vi "ConvertErrorToPLCMBits.vi"(11 "Error message":string) -> (2 "PLC message":string, 3 "Send?":bool)   [LabVIEW 2025]
uses:
  <vilib>/Utility/error.llb/Trim Whitespace One-Sided.vi
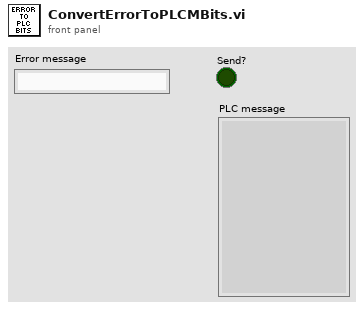
[diagram p1: front panel]
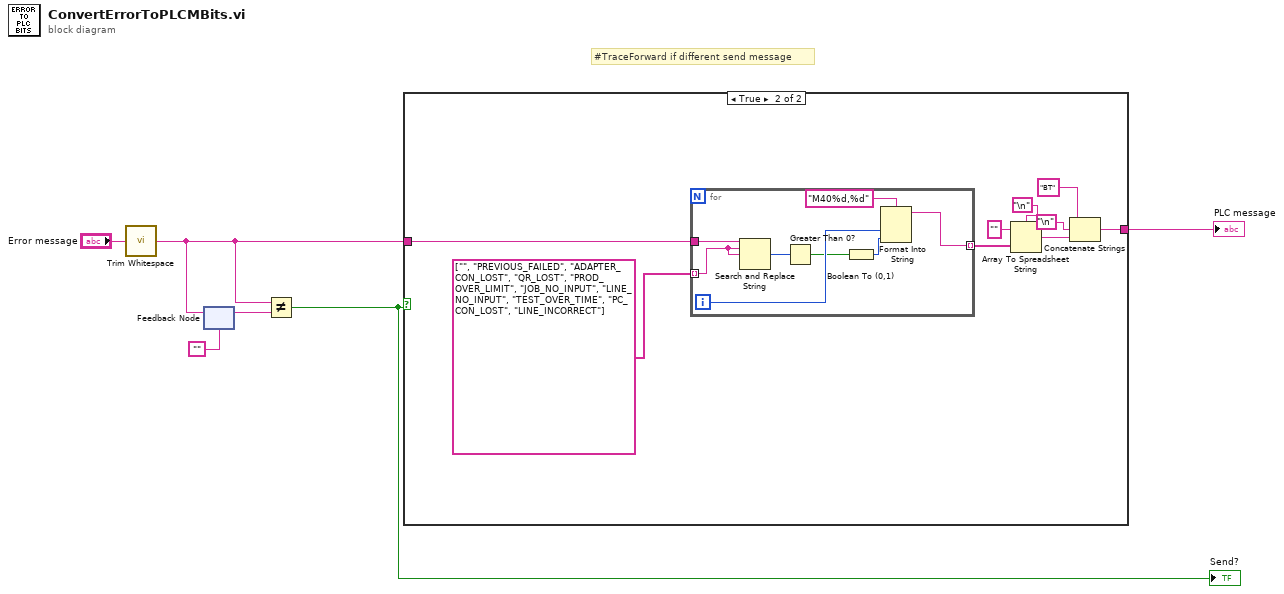
[diagram p0: block diagram]
diagram:
  # "#TraceForward if different send message"
  n1 = call <vilib>:"Trim Whitespace.vi"("string"="Error message") -> ("trimmed string"=w4:string)  [unwired: 1 in]
  n2 = feedback-in #1(w4) -> ()
  n3 = feedback #1("") -> (w6:string)
  n4 = Not Equal?(x=w4, y=w6) -> (x != y?=w3:bool)
  "Send?" <- w3
  n5 = case shown="True" w3 {
    tunnel: w4 -> [_ w15]
    tunnel: [_ w8] -> w2
    frame False {
    }
    frame True {
      n6 = for {
        tunnel: w15 -> [w23]
        tunnel: string[] ["", "PREVIOUS_FAILED", "ADAPTER_CON_LOST", "QR_LOST", "PROD_OVER_LIMIT", "JOB_NO_INPUT", "LINE_NO_INPUT", "TEST_OVER_TIME", "PC_CON_LOST", "LINE_INCORRECT"] -> [w22] mode=indexing
        tunnel: [w16] -> w13 mode=indexing
        i -> [w19]
        n7 = Search and Replace String(input string=w23, search string=w22, replace string=w22) -> (number of replacements=w21:i32)  [unwired: 5 in, 3 out]
        n8 = Greater Than 0?(x=w21) -> (x > 0?=w18:bool)
        n9 = Boolean To (0,1)(Boolean=w18) -> (0, 1=w17:i16)
        n10 = Format Into String(format string="M40%d,%d", w19, w17) -> (resulting string=w16:string)  [unwired: 2 in, 1 out]
      }
      n11 = Array To Spreadsheet String(delimiter (Tab)="\n", array=w13, 3:"" ("format string")) -> (spreadsheet string=w12:string)
      n12 = Concatenate Strings("BT" ("string"), "\n", w12) -> (w8:string)
    }
  }
  "PLC message" <- w2
